vi "Rule_Count_Direction.vi"(8 "error in":errorcluster, 9 "Direction":cluster{"dR":i32, "dC":i32}={"dR"=0, "dC"=1}, 10 "Move":T1={"Row"=7, "Col"=7, "Stone"=enum."Black"}, 11 "Grid":enum8{"Empty", "Black", "White"}[][](array[ring])=[[enum."Empty", enum."Empty", enum."Empty", enum."Empty", enum."Empty", enum."Empty", enum."Empty", enum."Empty", enum."Empty", enum."Empty", enum."Empty", enum."Empty", enum."Empty", enum."Empty", enum."Empty"], [enum."Empty", enum."Empty", enum."Empty", enum."Empty", enum."Empty", enum."Empty", enum."Empty", enum."Empty", enum."Empty", enum."Empty", enum."Empty", enum."Empty", enum."Empty", enum."Empty", enum."Empty"], [enum."Empty", enum."Empty", enum."Empty", enum."Empty", enum."Empty", enum."Empty", enum."Empty", enum."Empty", enum."Empty", enum."Empty", enum."Empty", enum."Empty", enum."Empty", enum."Empty", enum."Empty"], [enum."Empty", enum."Empty", enum."Empty", enum."Empty", enum."Empty", enum."Empty", enum."Empty", enum."Empty", enum."Empty", enum."Empty", enum."Empty", enum."Empty", enum."Empty", enum."Empty", enum."Empty"], [enum."Empty", enum."Empty", enum."Empty", enum."Empty", enum."Empty", enum."Empty", enum."Empty", enum."Empty", enum."Empty", enum."Empty", enum."Empty", enum."Empty", enum."Empty", enum."Empty", enum."Empty"], [enum."Empty", enum."Empty", enum."Empty", enum."Empty", enum."Empty", enum."Empty", enum."Empty", enum."Empty", enum."Empty", enum."Empty", enum."Empty", enum."Empty", enum."Empty", enum."Empty", enum."Empty"], [enum."Empty", enum."Empty", enum."Empty", enum."Empty", enum."Empty", enum."Empty", enum."Empty", enum."Empty", enum."Empty", enum."Empty", enum."Empty", enum."Empty", enum."Empty", enum."Empty", enum."Empty"], [enum."Empty", enum."Empty", enum."Empty", enum."Empty", enum."Empty", enum."Empty", enum."Empty", enum."Empty", enum."Empty", enum."Empty", enum."Empty", enum."Empty", enum."Empty", enum."Empty", enum."Empty"], [enum."Empty", enum."Empty", enum."Empty", enum."Empty", enum."Empty", enum."Empty", enum."Empty", enum."Empty", enum."Empty", enum."Empty", enum."Empty", enum."Empty", enum."Empty", enum."Empty", enum."Empty"], [enum."Empty", enum."Empty", enum."Empty", enum."Empty", enum."Empty", enum."Empty", enum."Empty", enum."Empty", enum."Empty", enum."Empty", enum."Empty", enum."Empty", enum."Empty", enum."Empty", enum."Empty"], [enum."Empty", enum."Empty", enum."Empty", enum."Empty", enum."Empty", enum."Empty", enum."Empty", enum."Empty", enum."Empty", enum."Empty", enum."Empty", enum."Empty", enum."Empty", enum."Empty", enum."Empty"], [enum."Empty", enum."Empty", enum."Empty", enum."Empty", enum."Empty", enum."Empty", enum."Empty", enum."Empty", enum."Empty", enum."Empty", enum."Empty", enum."Empty", enum."Empty", enum."Empty", enum."Empty"], [enum."Empty", enum."Empty", enum."Empty", enum."Empty", enum."Empty", enum."Empty", enum."Empty", enum."Empty", enum."Empty", enum."Empty", enum."Empty", enum."Empty", enum."Empty", enum."Empty", enum."Empty"], [enum."Empty", enum."Empty", enum."Empty", enum."Empty", enum."Empty", enum."Empty", enum."Empty", enum."Empty", enum."Empty", enum."Empty", enum."Empty", enum."Empty", enum."Empty", enum."Empty", enum."Empty"], [enum."Empty", enum."Empty", enum."Empty", enum."Empty", enum."Empty", enum."Empty", enum."Empty", enum."Empty", enum."Empty", enum."Empty", enum."Empty", enum."Empty", enum."Empty", enum."Empty", enum."Empty"]]) -> (0 "error out":errorcluster, 2 "Open End":bool, 3 "Count":i32)   [LabVIEW 2026]
doc: "Move 위치에서 Direction(dR,dC) 방향으로 같은 색 돌이 몇 개 연속되는지 센다(시작 칸 제외).\nOpen End = 연속이 끝난 다음 칸이 보드 안의 빈 칸이면 True."
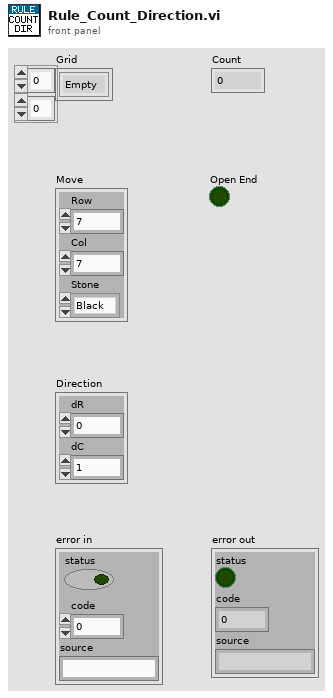
[diagram p1: front panel]
types:
  T1 = cluster{"Row":i32, "Col":i32, "Stone":enum8{"Empty", "Black", "White"}}
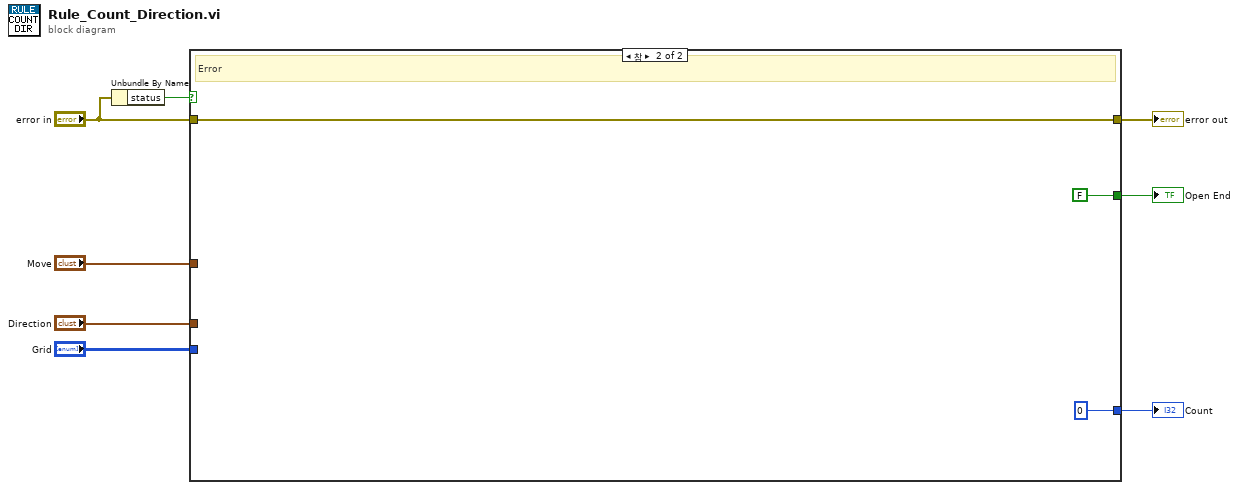
[diagram p0: block diagram]
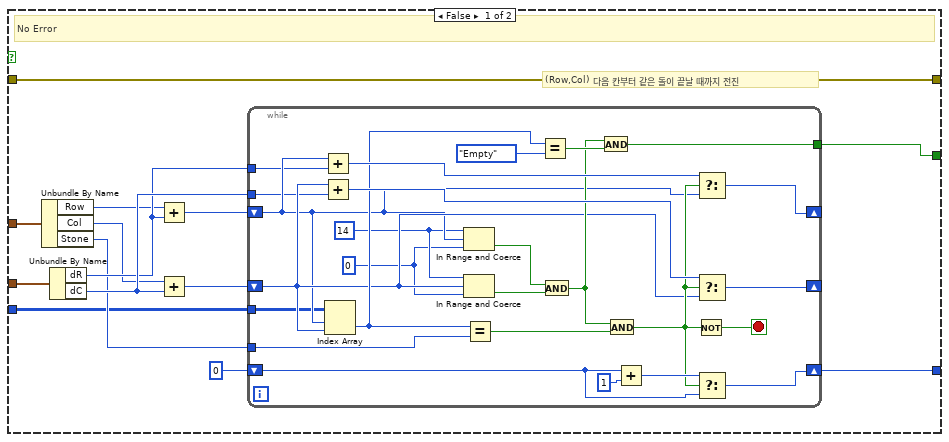
[diagram p2: hidden frame]
diagram:
  n1 = Unbundle By Name("error in") -> ("status"=w5:bool)
  n2 = case shown="참" w5 {
    tunnel: "Grid" -> [w9 _]
    tunnel: "Move" -> [w10 _]
    tunnel: "Direction" -> [w11 _]
    tunnel: "error in" -> [w12 w49]
    tunnel: [w22 0] -> w6
    tunnel: [w12 w49] -> w8
    tunnel: [w21 FALSE] -> w7
    frame False {
      # "(Row,Col) 다음 칸부터 같은 돌이 끝날 때까지 전진"
      # "No Error"
      n3 = Unbundle By Name(w10) -> ("Row"=w13:i32, "Col"=w14:i32, "Stone"=w15:enum8{"Empty", "Black", "White"})
      n4 = Unbundle By Name(w11) -> ("dR"=w16:i32, "dC"=w17:i32)
      n5 = Add(x=w13, y=w16) -> (x+y=w18:i32)
      n6 = Add(x=w14, y=w17) -> (x+y=w19:i32)
      n7 = while {
        shift-right: [w47] -> w22
        shift-left: 0 -> [w46]
        tunnel: w9 -> [w23]
        tunnel: w16 -> [w24]
        tunnel: w17 -> [w25]
        tunnel: w15 -> [w26]
        shift-right: [w42] -> _
        shift-left: w18 -> [w30]
        shift-right: [w44] -> _
        shift-left: w19 -> [w32]
        tunnel: [w39] -> w21
        stop <- w48 stop-if-true
        w28 = 14
        w27 = 0
        n8 = Add(x=w30, y=w24) -> (x+y=w41:i32)
        n9 = Add(x=w32, y=w25) -> (x+y=w43:i32)
        n10 = Index Array(array=w23, index (row)=w30, index (col)=w32) -> (element=w34:enum8{"Empty", "Black", "White"})
        n11 = In Range and Coerce(upper limit=w28, x=w30, lower limit=w27) -> (In Range?=w29:bool)  [unwired: 1 out]
        n12 = In Range and Coerce(upper limit=w28, x=w32, lower limit=w27) -> (In Range?=w31:bool)  [unwired: 1 out]
        n13 = Equal?(x=w34, y=w26) -> (x = y?=w35:bool)
        n14 = Equal?(x=w34, y=enum8{"Empty", "Black", "White"}."Empty") -> (x = y?=w38:bool)
        n15 = And(x=w29, y=w31) -> (x .and. y?=w33:bool)
        n16 = And(x=w33, y=w38) -> (x .and. y?=w39:bool)
        n17 = And(x=w33, y=w35) -> (x .and. y?=w36:bool)
        n18 = Add(x=w46, y=1) -> (x+y=w45:i32)
        n19 = Not(x=w36) -> (.not. x?=w48:bool)
        n20 = Select(t=w41, s=w36, f=w30) -> (s? t:f=w42:i32)
        n21 = Select(t=w43, s=w36, f=w32) -> (s? t:f=w44:i32)
        n22 = Select(t=w45, s=w36, f=w46) -> (s? t:f=w47:i32)
      }
    }
    frame True {
      # "Error"
    }
  }
  "Count" <- w6
  "Open End" <- w7
  "error out" <- w8
